vi "Launch Async Loop.vi"(8 "error in (no error)":errorcluster, 9 "Redraw Period":dbl, 10 "Has Local":bool, 11 "LocalGraphBuffer in":refnum<class "LocalGraphBuffer.lvclass">) -> (0 "error out":errorcluster, 3 "LocalGraphBuffer out":refnum<class "LocalGraphBuffer.lvclass">)   [LabVIEW 2020, in "VolatusGUIElements.lvlib" / "LocalGraphBuffer.lvclass"]
uses:
  LocalGraphBuffer.lvclass
  Buffer Redraw Async.vi
  LocalGraphBuffer.lvclass/LocalGraphBuffer.ctl
  Local Buffer Loop Async.vi
  lv-exec-anchor/ExecAnchor/ExecAnchor.lvclass
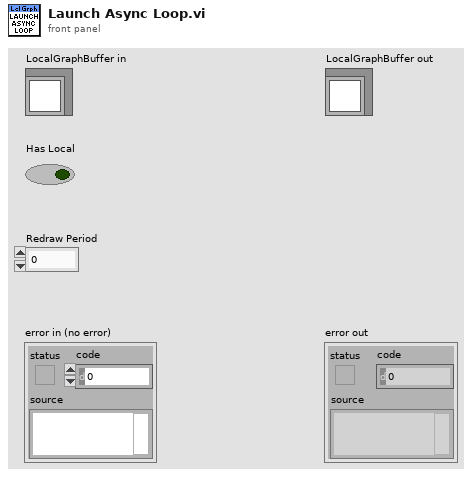
[diagram p1: front panel]
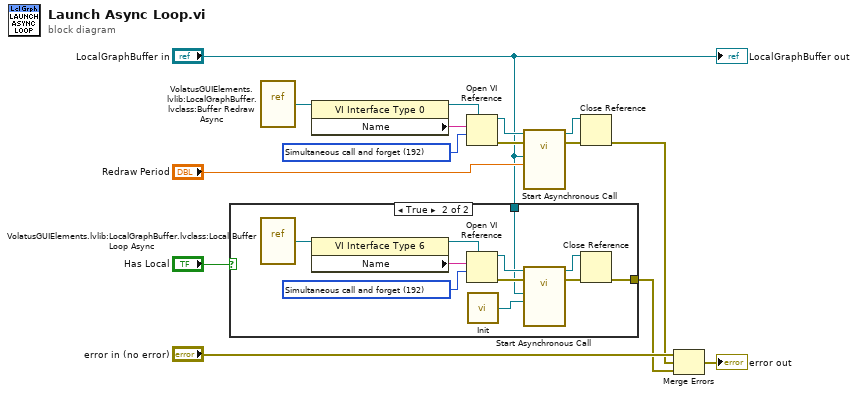
[diagram p0: block diagram]
diagram:
  w9 = 192 items=["Record modifications"=1, "Open templates for editing"=2, "Prompt user to save"=4, "Prepare for reentrant run"=8, "Prompt to find missing subVIs"=16, "Hide loading dialog box"=32, "Enable simultaneous calls"=64, "Prepare to call and forget"=128, "Simultaneous call and forget"=192, "Prepare to call and collect"=256, "Simultaneous call and collect"=320]
  n1 = case shown="True" "Has Local" {
    tunnel: "LocalGraphBuffer in" -> [_ w18]
    tunnel: [_ w17] -> w1
    frame False {
    }
    frame True {
      w24 = 192 items=["Record modifications"=1, "Open templates for editing"=2, "Prompt user to save"=4, "Prepare for reentrant run"=8, "Prompt to find missing subVIs"=16, "Hide loading dialog box"=32, "Enable simultaneous calls"=64, "Prepare to call and forget"=128, "Simultaneous call and forget"=192, "Prepare to call and collect"=256, "Simultaneous call and collect"=320]
      n2 = vi-ref "VolatusGUIElements.lvlib:LocalGraphBuffer.lvclass:Local Buffer Loop Async.vi"() -> (w26:refnum<vi>)
      n3 = property class="VI Interface Type 6"(reference=w26) -> (reference out=w23:refnum<vi>, "Name"=w25:string)  [unwired: 1 in, 1 out]
      n4 = Open VI Reference(type specifier VI Refnum (for type only)=w23, vi path=w25, options=w24) -> (vi reference=w21:refnum<vi>, error out=w22:errorcluster)  [unwired: 3 in]
      n5 = call "Init.vi"() -> ("ExecAnchor out"=w16:refnum<class "ExecAnchor.lvclass">)  [unwired: 7 in]
      n6 = call-by-ref "Start Asynchronous Call"(reference=w21, error in=w22, "ExecAnchor"=w16, "LocalGraphBuffer in"=w18) -> (reference out=w19:refnum<vi>, error out=w20:errorcluster)  [unwired: 10 in]
      n7 = Close Reference(reference=w19, error in (no error)=w20) -> (error out=w17:errorcluster)
    }
  }
  n8 = vi-ref "VolatusGUIElements.lvlib:LocalGraphBuffer.lvclass:Buffer Redraw Async.vi"() -> (w7:refnum<vi>)
  n9 = property class="VI Interface Type 0"(reference=w7) -> (reference out=w10:refnum<vi>, "Name"=w8:string)  [unwired: 1 in, 1 out]
  n10 = Open VI Reference(type specifier VI Refnum (for type only)=w10, vi path=w8, options=w9) -> (vi reference=w12:refnum<vi>, error out=w11:errorcluster)  [unwired: 3 in]
  n11 = call-by-ref "Start Asynchronous Call"(reference=w12, error in=w11, "Period s"="Redraw Period", "LocalGraphBuffer in"="LocalGraphBuffer in") -> (reference out=w14:refnum<vi>, error out=w13:errorcluster)  [unwired: 10 in]
  n12 = Close Reference(reference=w14, error in (no error)=w13) -> (error out=w5:errorcluster)
  n13 = Merge Errors("error in (no error)", w5, w1) -> (→"error out":errorcluster)
  "LocalGraphBuffer out" <- "LocalGraphBuffer in"
